vi "propnode_config.vi"() -> ()   [LabVIEW 2014]
panel:
  in  "Property Node Class Name":string
  in  "error in (no error)":errorcluster
  in  "reference":refnum<vi>
  out "reference out 2":refnum<vi>
  in  "Allow Alternate Names? (F)":bool
  in  "ID Strings[]":string[](array[string])
  in  "index":i32
  out "error out":errorcluster
  out "reference out":refnum<vi>
  in  "Is Write":bool
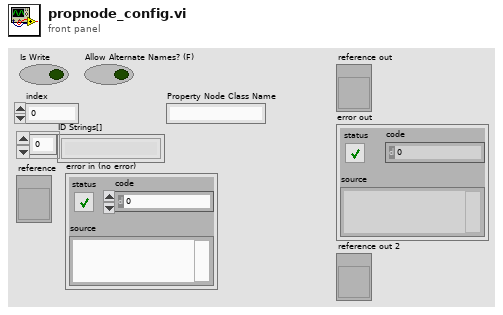
[diagram p1: front panel]
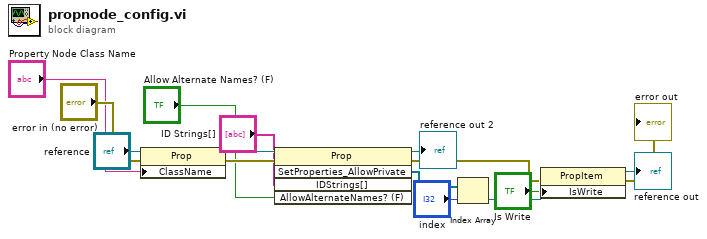
[diagram p0: block diagram]
diagram:
  n1 = property class="Prop"(reference="reference", error in="error in (no error)", "ClassName"="Property Node Class Name") -> (reference out=w15:refnum<vi>, error out=w14:errorcluster)
  n2 = invoke class="Prop" method="SetProperties_AllowPrivate"(reference=w15, error in=w14, "IDStrings[]"="ID Strings[]", "AllowAlternateNames? (F)"="Allow Alternate Names? (F)") -> (reference out=→"reference out 2":refnum<vi>, error out=w11:errorcluster, "SetProperties_AllowPrivate"=w13:refnum<vi>[])  [unwired: 1 in, 2 out]
  n3 = Index Array(array=w13, index="index") -> (element=w12:refnum<vi>)
  n4 = property class="PropItem"(reference=w12, error in=w11, "IsWrite"="Is Write") -> (reference out=→"reference out":refnum<vi>, error out=→"error out":errorcluster)
